vi "ResetArm.vi"(0 "Power/Speed 1":i8=-10, 1 "NXT/EV3 IN":T1, 2 "ResetTo":i32) -> (3 "NXT/EV3 OUT":T1)   [LabVIEW 2016, in "13.03 Robot.lvrbt"]
uses:
  13.03 Robot.lvrbt
  <vilib>/NXT/Subs/LVHSConnector.ctl
  <vilib>/NXT/LegoClasses/BrickReference/BrickReference.lvclass
  <vilib>/NXT/Block Support/NXT_OutputPort.ctl
  <vilib>/NXT/NXTIO Xnodes/NXTIONodeSubVIs/NXTMoveMotors.vi
  <vilib>/NXT/NXTIO Xnodes/NXTIONodeSubVIs/LEGOMotorStatus.vi
  <vilib>/NXT/NXTIO Xnodes/AddressXNode/NXTIOAddress.xnode
  <vilib>/NXT/NXTIO Xnodes/NXTIOXNode/NXTIO.xnode
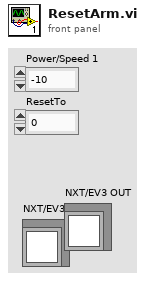
[diagram p1: front panel]
types:
  T1 = typedef "LVHSConnector.ctl" = refnum<class "BrickReference.lvclass">
  T2 = typedef "NXT_OutputPort.ctl" = u8
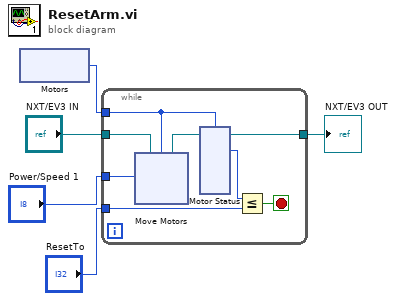
[diagram p0: block diagram]
diagram:
  n1 = xnode "Motors"() -> ("Motor"=w5:T2)
  n2 = while {
    tunnel: w5 -> [w11]
    tunnel: "Power/Speed 1" -> [w13]
    tunnel: "NXT/EV3 IN" -> [w12]
    tunnel: [w8] -> w2
    tunnel: "ResetTo" -> [w6]
    stop <- w7 stop-if-true
    n3 = xnode "Move Motors"("Power/Speed 1"=w13, "Motors"=w11, "NXT/EV3"=w12) -> ("NXT/EV3"=w10:T1)
    n4 = xnode "Motor Status"("Motors"=w11, "NXT/EV3"=w10) -> ("Position 1"=w9:i32, "NXT/EV3"=w8:T1)  [unwired: 1 out]
    n5 = Less Or Equal?(x=w9, y=w6) -> (x <= y?=w7:bool)
  }
  "NXT/EV3 OUT" <- w2
